vi "Test App Get Process Returns Self.vi"(8 "error in (no error)":errorcluster, 11 "Rig Test in":refnum<class "Application Dev Test.lvclass">) -> (0 "error out":errorcluster, 3 "Rig Test out":refnum<class "Application Dev Test.lvclass">)   [LabVIEW 2020, in "Application Dev Test.lvclass"]
uses:
  Application Dev Test.lvclass
  Application Dev Test.lvclass/Application Dev Test.ctl
  <vilib>/Astemes/LUnit/Test Case.lvclass
  source/Framework/Application/Application.lvclass
  source/Framework/Process/Process.lvclass
  C:/git/astemes-triarc-framework/source/Framework/Process/Process.lvclass
  C:/git/astemes-triarc-framework/source/Framework/Base/Base.lvclass
  C:/git/astemes-triarc-framework/source/Framework/Error Handler Interface/Error Handler Interface.lvclass
  C:/git/astemes-triarc-framework/source/Framework/Logging/Logging.lvclass
  C:/git/astemes-triarc-framework/source/Framework/Application/Application.lvclass
  C:/git/astemes-triarc-framework/source/Framework/Async Handler/Async Handler.lvclass
  C:/git/astemes-triarc-framework/source/Framework Test Suite/Process Test/Process Test.lvclass
  C:/git/astemes-triarc-framework/source/Framework Test Suite/Base Class Test/Base Test.lvclass
  C:/Program Files (x86)/National Instruments/LabVIEW 2020/vi.lib/Astemes/LUnit Test Inheritance/LUnit Inheriting Test Case.lvclass
  C:/Program Files (x86)/National Instruments/LabVIEW 2020/vi.lib/Astemes/LUnit/Test Case.lvclass
  C:/Program Files (x86)/National Instruments/LabVIEW 2020/vi.lib/Astemes/LUnit/LUnit Runnable.lvclass
  C:/git/astemes-triarc-framework/tests/Application Dev Test/Application Dev Test.lvclass
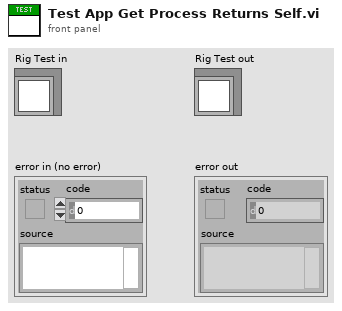
[diagram p1: front panel]
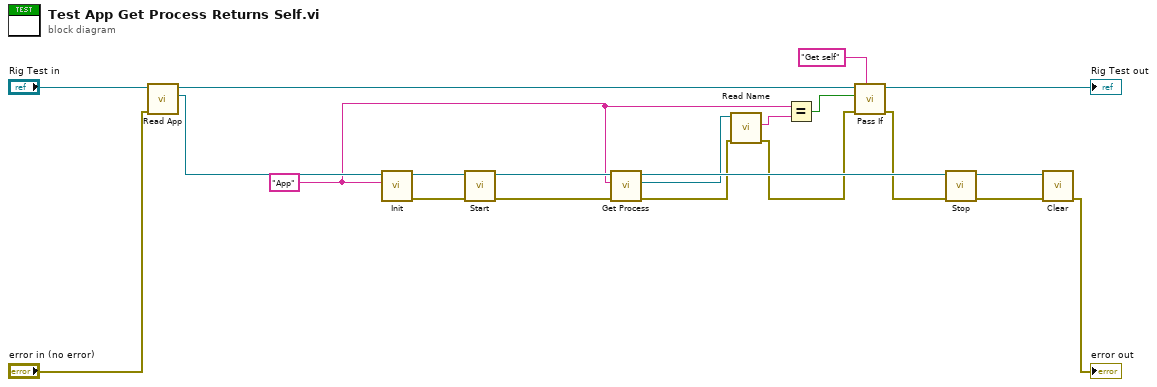
[diagram p0: block diagram]
diagram:
  w2 = "App" ("Name")
  n1 = call "Read App.vi"("error in (no error)"="error in (no error)", "Application Test In"="Rig Test in") -> ("App out"=w20:refnum<class "Application.lvclass">, "Application Test Out"=w9:refnum<class "Application Dev Test.lvclass">)  [unwired: 7 in, 1 out]
  n2 = call-dynamic "Init.vi"("Name"=w2, "Process In"=w20) -> ("error out"=w10:errorcluster, "Process Out"=w11:refnum<class "Application.lvclass">)  [unwired: 8 in]
  n3 = call "Start.vi"("error in (no error)"=w10, "Process In"=w11) -> ("error out"=w12:errorcluster, "Process Out"=w13:refnum<class "Application.lvclass">)  [unwired: 7 in, 1 out]
  n4 = call "Get Process.vi"("error in (no error)"=w12, "Process Name"=w2, "Application In"=w13) -> ("error out"=w4:errorcluster, "App Process"=w17:refnum<class "Process.lvclass">, "Application Out"=w18:refnum<class "Application.lvclass">)  [unwired: 6 in]
  n5 = call "Read Name.vi"("error in (no error)"=w4, "Process In"=w17) -> ("error out"=w3:errorcluster, "Qualified Name"=w5:string)  [unwired: 6 in, 2 out]
  n6 = Equal?(x=w2, y=w5) -> (x = y?=w14:bool)
  n7 = call <vilib>:"Pass If.vi"("Description"="Get self", "error in (no error)"=w3, "Pass?"=w14, "LUnit Test Case In"=w9) -> ("error out"=w15:errorcluster, "LUnit Test Case Out"=→"Rig Test out":refnum<class "Application Dev Test.lvclass">)  [unwired: 6 in]
  n8 = call "Stop.vi"("error in (no error)"=w15, "Process In"=w18) -> ("error out"=w8:errorcluster, "Process Out"=w7:refnum<class "Application.lvclass">)  [unwired: 7 in, 1 out]
  n9 = call-dynamic "Clear.vi"("error in (no error)"=w8, "Application In"=w7) -> ("error out"=→"error out":errorcluster)  [unwired: 9 in]
